vi "vi_get_callers.vi"(10 "VI":refnum<class "HierarchyNode.lvclass">, 11 "VIGraph in":refnum<class "HierarchyGraph.lvclass">) -> (1 "Callers":refnum<class "HierarchyNode.lvclass">[](array[class]), 2 "VI not found?":bool)   [LabVIEW 2020, in "vi-hierarchy.lvlib" / "HierarchyGraph.lvclass"]
uses:
  HierarchyGraph.lvclass
  VINode/HierarchyNode.lvclass
  C:/Projects/labview-project-load-tools/source/submodules/graph-api-labview/source/api/Node/Node.lvclass
  HierarchyGraph.lvclass/HierarchyGraph.ctl
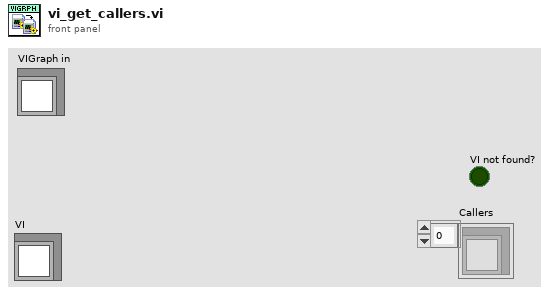
[diagram p1: front panel]
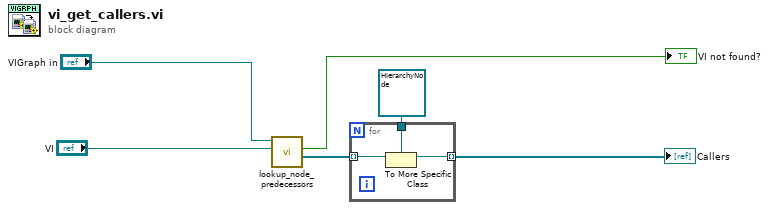
[diagram p0: block diagram]
diagram:
  n1 = call-dynamic "lookup_node_predecessors.vi"("node"="VI", "digraph"="VIGraph in") -> ("predecessors"=w1:refnum<class "Node.lvclass">[], "node not found?"=→"VI not found?":bool)  [unwired: 8 in]
  n2 = for {
    tunnel: w1 -> [w9] mode=indexing
    tunnel: [w8] -> w4 mode=indexing
    tunnel: refnum<class "HierarchyNode.lvclass"> refnum ("VINode") -> [w7]
    n3 = To More Specific Class(target class=w7, reference=w9) -> (specific class reference=w8:refnum<class "HierarchyNode.lvclass">)  [unwired: 1 in, 1 out]
  }
  "Callers" <- w4
